vi "set Gate Enable.vi"(8 "error in (no error)":errorcluster, 10 "Gate Enable":bool, 11 "Keysight 9020A in":refnum<class "Keysight 9020A.lvclass">) -> (0 "error out":errorcluster, 3 "Keysight 9020A out":refnum<class "Keysight 9020A.lvclass">)   [LabVIEW 2023, in "Spectrum Analyzer.lvlib" / "Keysight 9020A.lvclass"]
uses:
  Keysight 9020A.lvclass
  Keysight 9020A.lvclass/Keysight 9020A.ctl
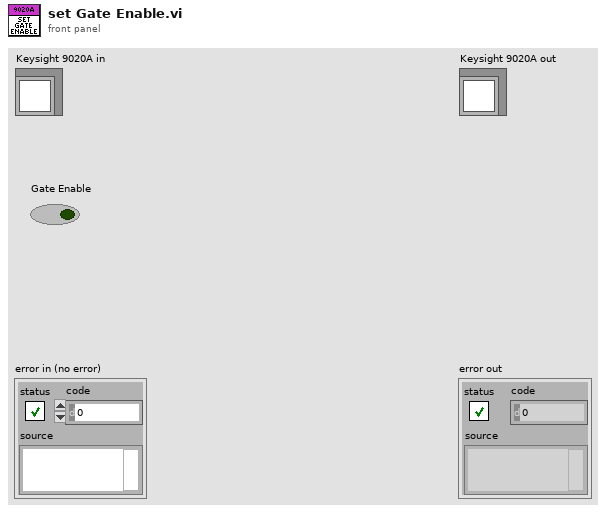
[diagram p1: front panel]
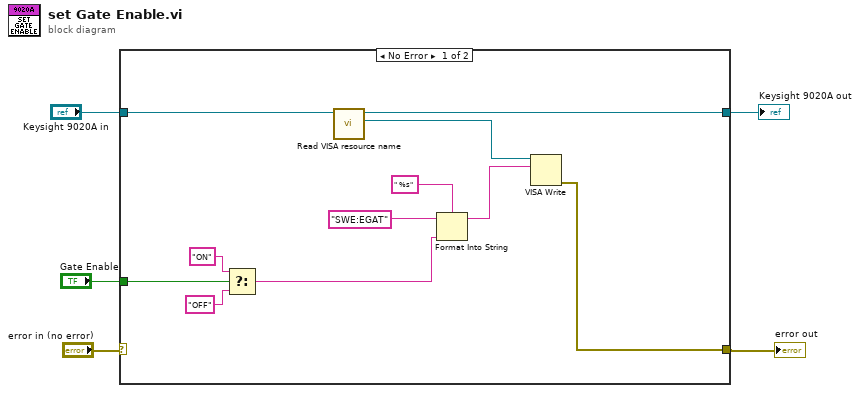
[diagram p0: block diagram]
diagram:
  n1 = case shown="No Error" "error in (no error)" {
    selector: "error in (no error)" -> [_ w17]
    tunnel: "Keysight 9020A in" -> [w11 w18]
    tunnel: [w16 w18] -> w4
    tunnel: [w12 w17] -> w1
    tunnel: "Gate Enable" -> [w7 _]
    frame No Error {
      n2 = Select(t="ON", s=w7, f="OFF") -> (s? t:f=w6:string)
      n3 = call "Read VISA resource name.vi"("Keysight 9020A in"=w11) -> ("VISA resource name"=w14:refnum<visa-resource-name>, "Keysight 9020A out"=w16:refnum<class "Keysight 9020A.lvclass">)  [unwired: 8 in, 1 out]
      n4 = Format Into String(format string=" %s", initial string="SWE:EGAT" ("string"), w6) -> (resulting string=w13:string)  [unwired: 1 in, 1 out]
      n5 = VISA Write(VISA resource name=w14, write buffer=w13) -> (error out=w12:errorcluster)  [unwired: 1 in, 2 out]
    }
    frame Error {
    }
  }
  "error out" <- w1
  "Keysight 9020A out" <- w4
